vi "QuickStartTemplate.vi"(11 "Error In":errorcluster) -> (15 "Error Out":errorcluster)   [LabVIEW 2016, in "Drona.lvlib"]
doc: "Template to start the initial steps for Drona Test"
uses:
  Drona.lvlib
  Stimulus/ControlValue/SetValueAuto.vi
  Assert/AssertControlValue/Equal.vi
  <vilib>/addons/_JKI Toolkits/Caraya/classes/Test/Test.lvclass
  Stimulus/ControlValue/ControlValue.lvlib
  Assert/AssertControlValue/AssertControlValue.lvlib
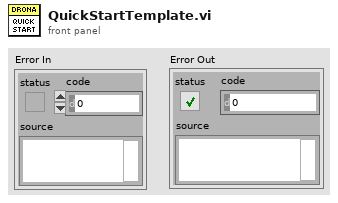
[diagram p1: front panel]
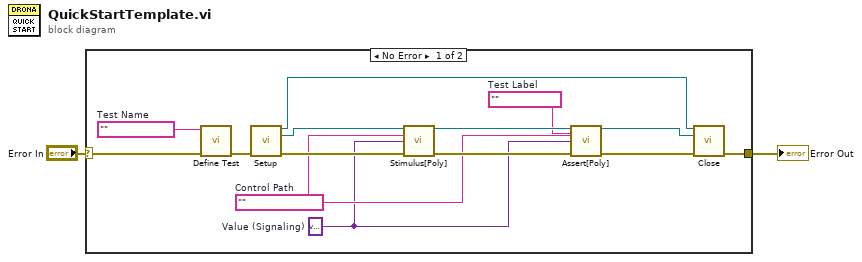
[diagram p0: block diagram]
diagram:
  n1 = case shown="No Error" "Error In" {
    selector: "Error In" -> [w15 w17]
    tunnel: [w3 w17] -> w1
    frame No Error {
      w5 = ""  # Test Label
      w8 = variant  # Value (Signaling)
      w9 = ""  # Control Path
      w16 = ""  # Test Name
      n2 = call <vilib>:"Define Test.vi"("error in (no error)"=w15, "Label (VI Title)"=w16) -> ("error out"=w14:errorcluster)  [unwired: 8 in, 1 out]
      n3 = call "Setup.vi"("error in"=w14) -> ("Application Ref"=w4:refnum<vi>, "VI Reference Out"=w12:refnum<vi>, "error out"=w13:errorcluster)  [unwired: 12 in]
      n4 = call-poly "Stimulus[Poly].vi"("VI Reference In"=w12, "Control Path"=w9, "Value (Signaling)"=w8, "error in"=w13) -> ("VI Reference Out"=w10:refnum<vi>, "error out"=w11:errorcluster)  [unwired: 10 in]
      n5 = call-poly "Assert[Poly].vi"("VI Reference In"=w10, "Test Label"=w5, "Control Path"=w9, "Control Value"=w8, "Error In"=w11) -> ("VI Reference Out"=w6:refnum<vi>, "Error Out"=w7:errorcluster)  [unwired: 8 in, 1 out]
      n6 = call "Close.vi"("Application Ref"=w4, "VI Reference"=w6, "error in"=w7) -> ("error out"=w3:errorcluster)  [unwired: 12 in]
    }
    frame Error {
    }
  }
  "Error Out" <- w1
